vi "Get path (absolute).vi"(6 "Strip lead \"/\" (F)":bool, 8 "error in (no error)":errorcluster, 9 "Encoded? (F)":bool, 11 "URI-Component.Path in":refnum<class "URI-Component.Path.lvclass">) -> (0 "error out":errorcluster, 2 "path-component":string, 3 "URI-Component.Path out":refnum<class "URI-Component.Path.lvclass">)   [LabVIEW 2013, in "openURI.lvlib" / "URI-Component.Path.lvclass"]
uses:
  URI-Component.Path.lvclass
  URI-Component.Path.lvclass/URI-Component.Path.ctl
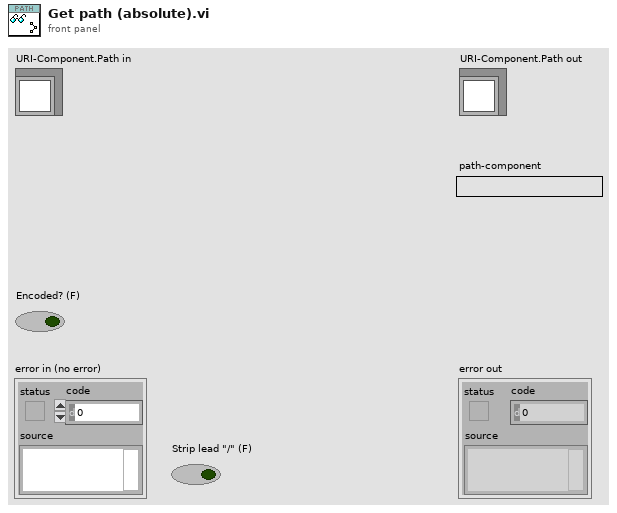
[diagram p1: front panel]
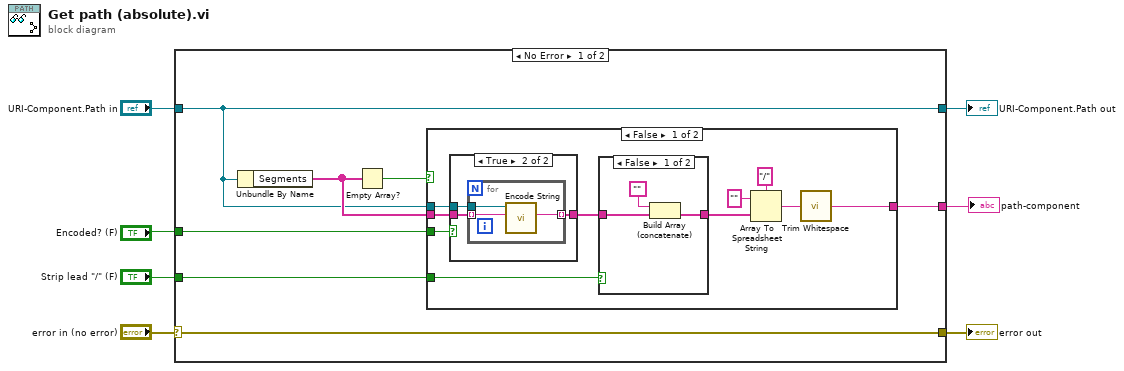
[diagram p0: block diagram]
diagram:
  n1 = case shown="No Error" "error in (no error)" {
    selector: "error in (no error)" -> [w14 w37]
    tunnel: [w14 w37] -> w6
    tunnel: [w10 w36] -> w4
    tunnel: "URI-Component.Path in" -> [w10 w36]
    tunnel: [w11 _] -> w3
    tunnel: "Encoded? (F)" -> [w9 _]
    tunnel: "Strip lead \"/\" (F)" -> [w8 _]
    frame No Error {
      n2 = Unbundle By Name(w10) -> ("Segments"=w12:string[])
      n3 = Empty Array?(array=w12) -> (empty?=w13:bool)
      n4 = case shown="False" w13 {
        tunnel: w12 -> [w19 _]
        tunnel: [w20 _] -> w11
        tunnel: w10 -> [w17 _]
        tunnel: w9 -> [w16 _]
        tunnel: w8 -> [w15 _]
        frame False {
          n5 = case shown="True" w16 {
            tunnel: w19 -> [w29 w32]
            tunnel: [w29 w31] -> w18
            tunnel: w17 -> [_ w30]
            frame False {
            }
            frame True {
              n6 = for {
                tunnel: w32 -> [w35] mode=indexing
                tunnel: [w34] -> w31 mode=indexing
                tunnel: w30 -> [w33]
                n7 = call-dynamic "Encode String.vi"("String"=w35, "URI-Component.Path"=w33) -> ("Encoded String"=w34:string)  [unwired: 9 in]
              }
            }
          }
          n8 = case shown="False" w15 {
            tunnel: [w26 w28] -> w21
            tunnel: w18 -> [w25 w28]
            frame False {
              n9 = Build Array (concatenate)("", w25) -> (w26:string[])
            }
            frame True {
            }
          }
          n10 = Array To Spreadsheet String(delimiter (Tab)="/", array=w21, 3:"" ("format string")) -> (spreadsheet string=w22:string)
          n11 = call <vilib>:"Trim Whitespace.vi"("string"=w22) -> ("trimmed string"=w20:string)  [unwired: 1 in]
        }
        frame True {
        }
      }
    }
    frame Error {
    }
  }
  "error out" <- w6
  "URI-Component.Path out" <- w4
  "path-component" <- w3
